vi "Module Init.vi"(8 "error in (no error)":errorcluster, 11 "GenericGuiAI in":refnum<class "GenericGuiAI.lvclass">) -> (0 "error out":errorcluster, 3 "GenericGuiAI out":refnum<class "GenericGuiAI.lvclass">)   [LabVIEW 2020, in "VolatusDAQGenericGUI.lvlib" / "GenericGuiAI.lvclass"]
uses:
  GenericGuiAI.lvclass
  C:/dev/lv20CE/relink/lv-volatus/Volatus/Module/Module.lvclass
  VolatusConfig/Meta Type.ctl
  VolatusConfig/Meta Name.ctl
  Volatus/Module/Module.lvclass/Module.ctl
  VolatusConfig/VolatusConfigElement/VolatusConfigElement.lvclass/VolatusConfigElement.ctl
  GenericGuiAI.lvclass/GenericGuiAI.ctl
  Volatus/Module/Config.vi
  VolatusConfig/VolatusConfigElement/Element.vi
  VolatusConfig/Task/Task Config.lvclass
  C:/dev/lv20CE/relink/lv-volatus/VolatusConfig/VolatusConfigElement/VolatusConfigElement.lvclass
  VolatusConfig/Cluster/Cluster Config.lvclass
  lv-cdm/CDM-Config/Config Lookup/Match Meta.vi
  lv-cdm/CDM-Config/Config Element/Owner.vi
  lv-cdm/CDM-Config/Config Manager/Lookup Descendant.vi
  VolatusConfig/Group/Group Config.lvclass
  lv-cdm/CDM-Config/Config Filter/Config Lookup.lvclass
  VolatusConfig/VolatusConfig.lvlib
  Volatus/Module/Module.lvclass
  VolatusConfig/Node/Node Config.lvclass
  VolatusConfig/VolatusConfigElement/VolatusConfigElement.lvclass
  lv-cdm/CDM-Config/Config Element/Config Element.lvclass
  C:/dev/lv20CE/relink/lv-volatus/VolatusDAQGenericGUI/GenericGuiAI/GenericGuiAI.lvclass
  C:/dev/lv20CE/relink/lv-volatus/VolatusConfig/Task/Task Config.lvclass
  C:/dev/lv20CE/relink/lv-volatus/VolatusConfig/Cluster/Cluster Config.lvclass
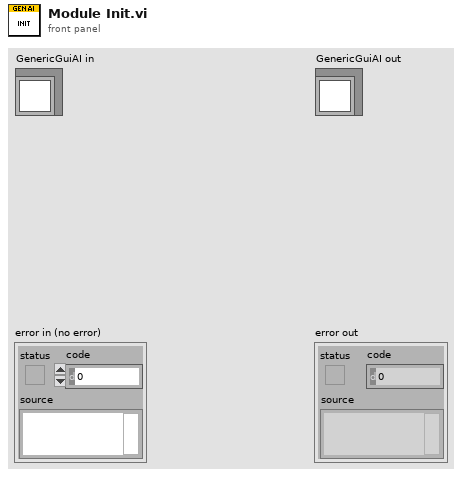
[diagram p1: front panel]
types:
  T1 = typedef "VolatusConfig.lvlib/Meta Name.ctl" = enum16{"VL_Type", "VL_Node_IP", "VL_Node_Type", "VL_Task_Type", "VL_Group_Type", "VL_Channel_Type", "VL_Channel_DataType", "VL_Config_Version", "VL_Overlay_Type", "VL_Config_Hash"}
  T2 = typedef "VolatusConfig.lvlib/Meta Type.ctl" = enum16{"UNKNOWN", "VL_System", "VL_Cluster", "VL_Node", "VL_Task", "VL_Group", "VL_Channel", "VL_Task_List", "VL_Scaling", "VL_Sensor", "VL_Sensor_List", "VL_Scale"}
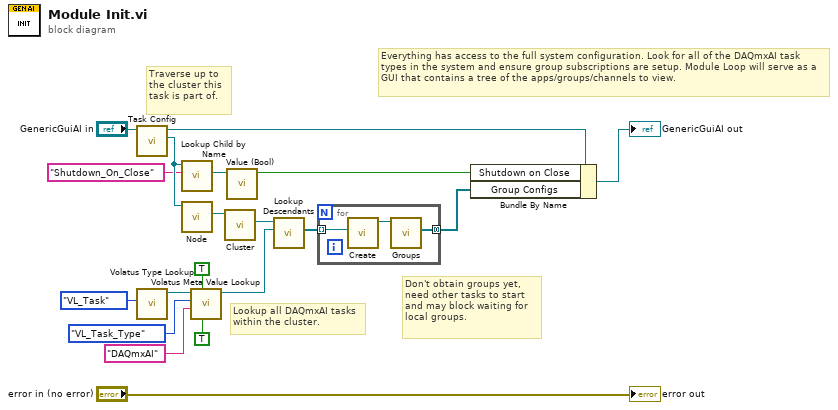
[diagram p0: block diagram]
diagram:
  # "Don't obtain groups yet, need other tasks to start and may block waiting for local groups."
  # "Lookup all DAQmxAI tasks within the cluster."
  # "Traverse up to the cluster this task is part of."
  # "Everything has access to the full system configuration. Look for all of the DAQmxAI task types in the system and ensure group subscriptions are setup. Module Loop will serve as a GUI that contains a tree of the apps/groups/channels to view."
  n1 = call "Task Config.vi"("Module in"="GenericGuiAI in") -> ("Task Config"=w4:refnum<class "Task Config.lvclass">, "Module out"=w12:refnum<class "GenericGuiAI.lvclass">)  [unwired: 8 in, 1 out]
  n2 = call "Volatus Type Lookup.vi"("Meta Type"=Meta_Type."VL_Task") -> ("Config Lookup out"=w17:refnum<class "Config Lookup.lvclass">)  [unwired: 9 in, 1 out]
  n3 = call "Lookup Child by Name.vi"("Child Name"="Shutdown_On_Close", "VolatusConfigElement in"=w4) -> ("Child"=w2:refnum<class "Config Element.lvclass">)  [unwired: 6 in, 3 out]
  n4 = call "Node.vi"("Task in"=w4) -> ("Node"=w8:refnum<class "Node Config.lvclass">)  [unwired: 8 in, 2 out]
  n5 = call "Volatus Meta Value Lookup.vi"("Exact Value (F)"=TRUE, "Don't Recurse Past Match (F)"=TRUE, "Value"="DAQmxAI", "Meta Name"=Meta_Name."VL_Task_Type", "Config Lookup (New)"=w17) -> ("Config Lookup out"=w6:refnum<class "Config Lookup.lvclass">)  [unwired: 5 in, 1 out]
  n6 = call "Cluster.vi"("Node in"=w8) -> ("Cluster"=w7:refnum<class "Cluster Config.lvclass">)  [unwired: 8 in, 2 out]
  n7 = call "Value (Bool).vi"("Config Element in"=w2) -> ("Bool Value"=w1:bool)  [unwired: 9 in, 1 out]
  n8 = call "Lookup Descendants.vi"("Lookup"=w6, "VolatusConfigElement in"=w7) -> ("Descendants"=w5:refnum<class "Config Element.lvclass">[])  [unwired: 7 in, 2 out]
  n9 = for {
    tunnel: w5 -> [w22] mode=indexing
    tunnel: [w20] -> w11 mode=concatenating
    n10 = call "Create.vi"("Element"=w22) -> ("Task out"=w21:refnum<class "Task Config.lvclass">)  [unwired: 9 in, 1 out]
    n11 = call "Groups.vi"("Task in"=w21) -> ("Groups"=w20:refnum<class "Group Config.lvclass">[])  [unwired: 8 in, 2 out]
  }
  n12 = Bundle By Name(cluster=w12, "Shutdown on Close"=w1, "Group Configs"=w11) -> (→"GenericGuiAI out":refnum<class "GenericGuiAI.lvclass">)
  "error out" <- "error in (no error)"
